vi "Host_Message_Loop.vi"(8 "error in (no error)":errorcluster={"status"=FALSE, "code"=0, "source"="\"\""}, 10 "app-state shift register":string, 11 "HostMessage.ctl queue":string) -> (0 "error out":errorcluster={"status"=FALSE, "code"=0, "source"="\"\""}, 2 "status ok":bool, 3 "HMI updates":string)   [LabVIEW 2026]
doc: "INTENT: Handle Host application commands. LOGIC: Dequeue commands and dispatch by enum; update Host state and send commands to selected target."
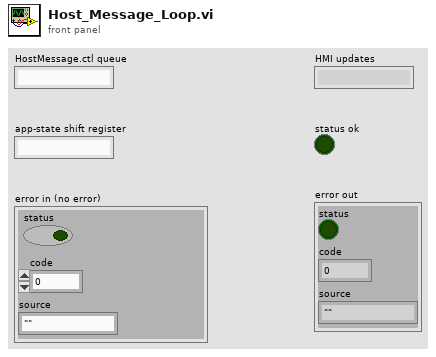
[diagram p1: front panel]
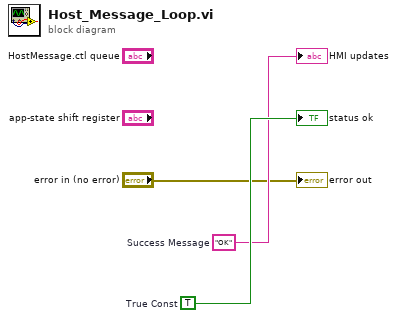
[diagram p0: block diagram]
diagram:
  w3 = TRUE  # True Const
  w2 = "OK"  # Success Message
  "HMI updates" <- w2
  "status ok" <- w3
  "error out" <- "error in (no error)"
